vi "Parameters File Handler.vi"(8 "error in":errorcluster, 10 "selected parameters file":path caption="path to parameters xml", 11 "configuration files page data in":T1 {"custom device ref" format="%.0x"}) -> (0 "error out":errorcluster, 3 "configuration files page data out":T1 {"custom device ref" format="%.0x"})   [LabVIEW 2026, in "AIM ARINC 429 System Explorer.lvlib" / "Implementation.lvlib"]
uses:
  Implementation.lvlib
  Import/ARINC 429 Import.lvlib
  Types/Browse Button.ctl
  Types/Path Control.ctl
  Scripting/AIM/AIM ARINC 429 Scripting.lvlib
  <vilib>/NI VeriStand/Custom Device API/Custom Device Item Ref.ctl
  <vilib>/NI VeriStand/Custom Device API/Custom Device API.lvlib
  Types/Configuration Files Page Data.ctl
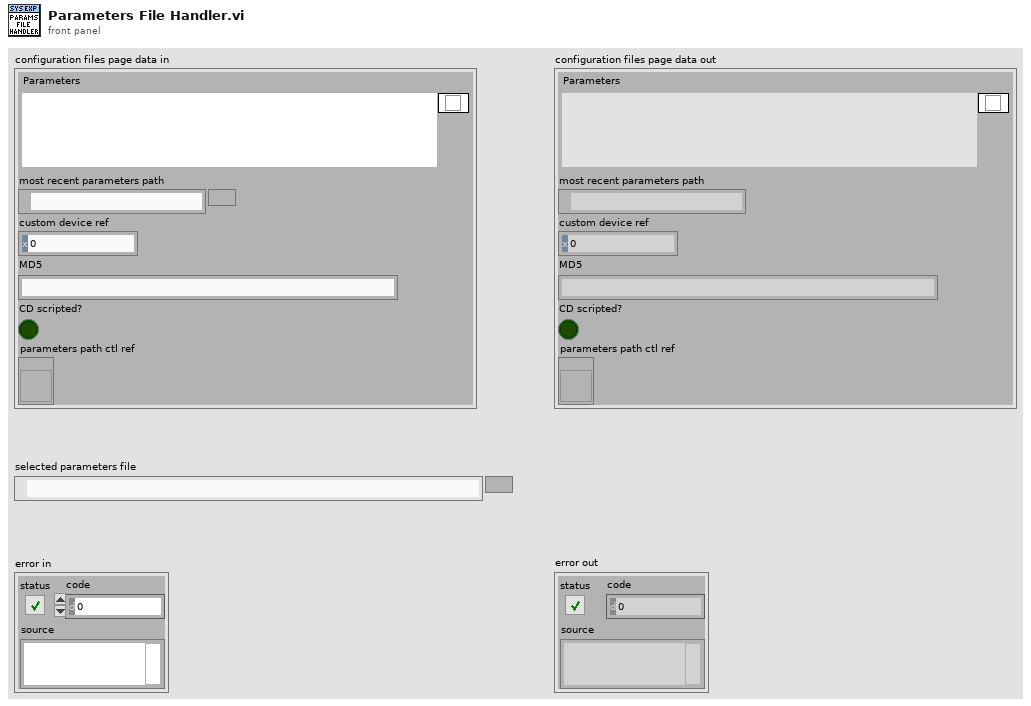
[diagram p1: front panel]
types:
  T1 = typedef "AIM ARINC 429 System Explorer.lvlib/Implementation.lvlib/Configuration Files Page Data.ctl" = cluster{"Parameters":T2, "most recent parameters path":path, "custom device ref":T4, "MD5":string, "CD scripted?":bool, "parameters path ctl ref":refnum<vi>}
  T2 = typedef "AIM ARINC 429 System Explorer.lvlib/Implementation.lvlib/Path Control.ctl" = cluster{"file path":path, "Browse":T3}
  T3 = typedef "AIM ARINC 429 System Explorer.lvlib/Implementation.lvlib/Browse Button.ctl" = bool
  T4 = typedef "Custom Device API.lvlib/Custom Device Item Ref.ctl" = u64
  T5 = typedef "VS Channels Definition for All Labels on Hardware Channel.ctl" = cluster{"hardware channel":i32, "direction":T6, "labels":T7[], "speed":T12}
  T6 = typedef "Direction.ctl" = enum16{"Rx", "Tx"}
  T7 = typedef "VS Channels Definition for Label.ctl" = cluster{"label (Dec)":u32, "parameters":T8[], "SDI value":u8, "SDI enabled":bool, "transfer type":T11, "create timestamp":bool, "transmit period":u32}
  T8 = typedef "VS Channel Definition for Parameter.ctl" = cluster{"name":string, "unit":string, "Parameter":T9}
  T9 = typedef "Parameter Definition.ctl" = cluster{"start index":i32, "size":i32, "encoding":T10, "signed":bool, "scale multiplier":dbl, "scale offset":dbl, "default value":dbl}
  T10 = typedef "Encoding and Decoding.lvlib/Encoding.ctl" = enum16{"BNR", "BCD", "Discrete"}
  T11 = typedef "Transfer Type.ctl" = enum16{"Scheduled", "Acyclic", "Block", "Strobe"}
  T12 = typedef "Transfer Speed.ctl" = enum16{"LO (12.5 kb/s)", "HI (100 kb/s)"}
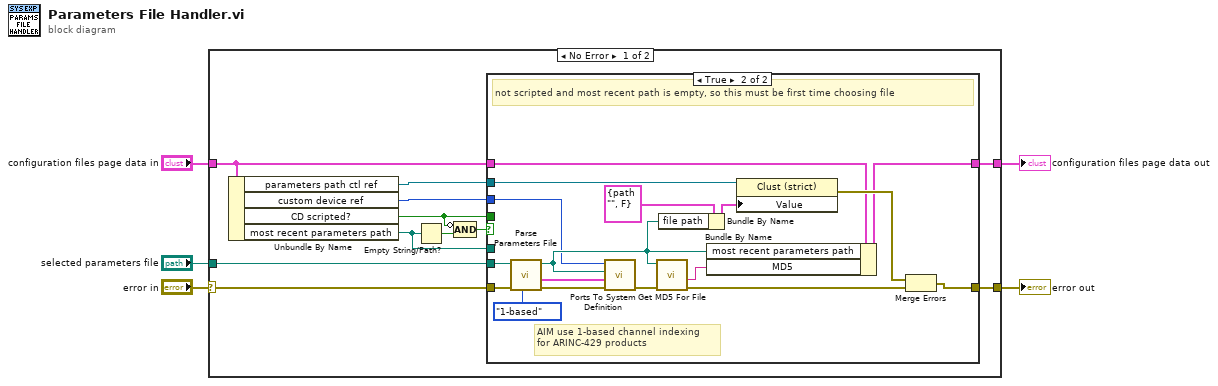
[diagram p0: block diagram]
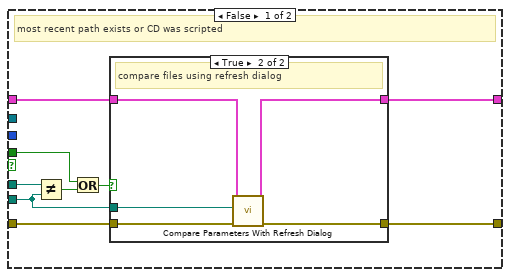
[diagram p2: hidden frame]
diagram:
  n1 = case shown="No Error" "error in" {
    selector: "error in" -> [w16 w51]
    tunnel: [w15 w51] -> w4
    tunnel: "configuration files page data in" -> [w13 w50]
    tunnel: [w12 w50] -> w2
    tunnel: "selected parameters file" -> [w14 _]
    frame No Error {
      n2 = Unbundle By Name(w13) -> ("parameters path ctl ref"=w6:refnum<vi>, "custom device ref"=w7:T4, "CD scripted?"=w8:bool, "most recent parameters path"=w11:path)
      n3 = Empty String/Path?(string/path=w11) -> (empty?=w10:bool)
      n4 = Compound Arithmetic op=AND(invert w8, w10) -> (w9:bool)
      n5 = case shown="True" w9 {
        tunnel: w16 -> [w25 w49]
        tunnel: w14 -> [w24 w48]
        tunnel: [w23 w43] -> w15
        tunnel: w11 -> [w22 _]
        tunnel: w13 -> [w21 w42]
        tunnel: [w20 w41] -> w12
        tunnel: w8 -> [w17 _]
        tunnel: w7 -> [_ w36]
        tunnel: w6 -> [_ w35]
        frame False {
          # "most recent path exists or CD was scripted"
          n6 = Not Equal?(x=w22, y=w24) -> (x != y?=w19:bool)
          n7 = Or(x=w17, y=w19) -> (x .or. y?=w18:bool)
          n8 = case shown="True" w18 {
            tunnel: w25 -> [w27 w32]
            tunnel: w24 -> [_ w28]
            tunnel: [w27 w29] -> w23
            tunnel: w21 -> [w26 w31]
            tunnel: [w26 w30] -> w20
            frame False {
              # "same path and CD not scripted, so do nothing"
            }
            frame True {
              # "compare files using refresh dialog"
              n9 = call "Compare Parameters With Refresh Dialog.vi"("error in"=w32, "selected parameters file"=w28, "configuration files page data in"=w31) -> ("error out"=w29:errorcluster, "configuration files page data out"=w30:T1)  [unwired: 7 in]
            }
          }
        }
        frame True {
          # "AIM use 1-based channel indexing\nfor ARINC-429 products"
          # "not scripted and most recent path is empty, so this must be first time choosing file"
          n10 = call "Parse Parameters File.vi"("ch indexing (0-based)"=enum16{"0-based", "1-based"}."1-based", "error in"=w49, "path to XML document"=w48) -> ("error out"=w47:errorcluster, "ports"=w46:T5[], "path to XML document out"=w38:path)  [unwired: 6 in]
          n11 = call "Ports To System Definition.vi"("error in"=w47, "ports"=w46, "parameter configuration file path"=w38, "custom device ref"=w36) -> ("error out"=w40:errorcluster)  [unwired: 6 in, 1 out]
          n12 = call "Get MD5 For File.vi"("error in"=w40, "path"=w38) -> ("error out"=w39:errorcluster, "MD5"=w37:string)  [unwired: 8 in]
          n13 = Bundle By Name(cluster=T2 {"file path"=path "", "Browse"=FALSE} ("Value"), "file path"=w38) -> (w34:T2)
          n14 = Bundle By Name(cluster=w42, "most recent parameters path"=w38, "MD5"=w37) -> (w41:T1)
          n15 = property class="Clust (strict)"(reference=w35, "Value"=w34) -> (error out=w44:errorcluster)  [unwired: 1 in, 1 out]
          n16 = Merge Errors(w44, w39) -> (w43:errorcluster)
        }
      }
    }
    frame Error {
    }
  }
  "error out" <- w4
  "configuration files page data out" <- w2
